vi "SaveFrontPanelImage.vi"(0 "VI Reference In":refnum<vi>, 5 "Image Store Path":path, 11 "Error In":errorcluster) -> (4 "VI Reference Out":refnum<vi>, 15 "Error Out":errorcluster)   [LabVIEW 2019, in "Drona.lvlib"]
doc: "This VI stores front panel of the given VI reference as an image to the given file path in png format"
uses:
  Drona.lvlib
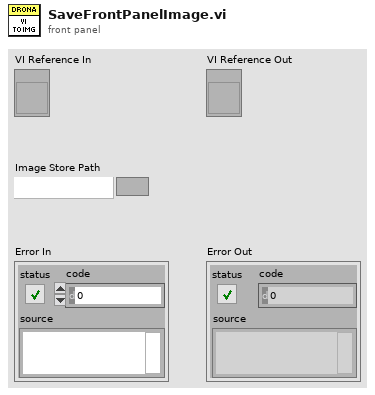
[diagram p1: front panel]
types:
  T1 = typedef "imagedata.ctl" = cluster{"image type":i32, "image depth":i32, "image":u8[], "mask":u8[], "colors":u32[], "Rectangle":cluster{"left":i16, "top":i16, "right":i16, "bottom":i16}}
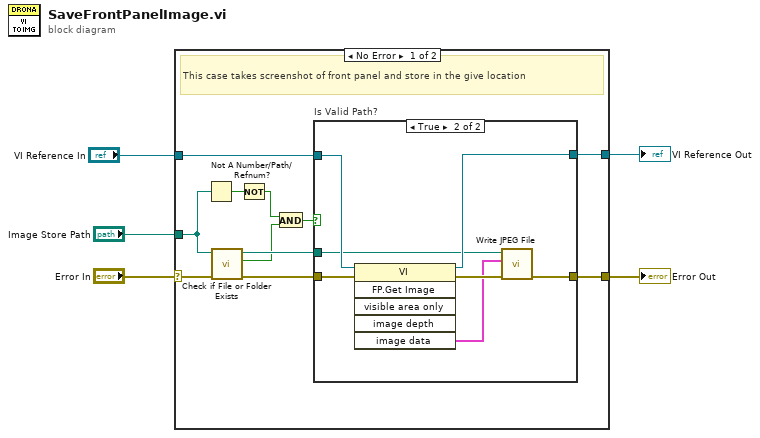
[diagram p0: block diagram]
diagram:
  n1 = case shown="No Error" "Error In" {
    selector: "Error In" -> [w12 w26]
    tunnel: "Image Store Path" -> [w10 _]
    tunnel: "VI Reference In" -> [w15 w27]
    tunnel: [w14 w27] -> w2
    tunnel: [w13 w26] -> w1
    frame No Error {
      # "This case takes screenshot of front panel and store in the give location"
      n2 = Not A Number/Path/Refnum?(number/path/refnum=w10) -> (NaN/Path/Refnum?=w16:bool)
      n3 = call <vilib>:"Check if File or Folder Exists.vi"("error in (no error)"=w12, "path"=w10) -> ("error out"=w11:errorcluster, "file or folder exists?"=w8:bool, "dup path"=w9:path)  [unwired: 7 in]
      n4 = Not(x=w16) -> (.not. x?=w7:bool)
      n5 = And(x=w7, y=w8) -> (x .and. y?=w6:bool)
      n6 = case "Is Valid Path?" shown="True" w6 {
        tunnel: w11 -> [w17 w25]
        tunnel: w15 -> [w18 w24]
        tunnel: w9 -> [_ w19]
        tunnel: [w18 w23] -> w14
        tunnel: [w17 w21] -> w13
        frame False {
        }
        frame True {
          n7 = invoke class="VI" method="FP.Get Image"(reference=w24, error in=w25) -> (reference out=w23:refnum<vi>, error out=w22:errorcluster, "image data"=w20:T1)  [unwired: 4 in, 3 out]
          n8 = call <vilib>:"Write JPEG File.vi"("error in (no error)"=w22, "image data"=w20, "path to JPEG file"=w19) -> ("error out"=w21:errorcluster)  [unwired: 7 in, 1 out]
        }
      }
    }
    frame Error {
      # "If error, this case pass that error message only"
    }
  }
  "Error Out" <- w1
  "VI Reference Out" <- w2
